vi "packet_build.vi"(9 "D2":u8, 10 "D1":u8, 11 "CMD":u8 format="%x") -> (3 "packet":string)   [LabVIEW 2026]
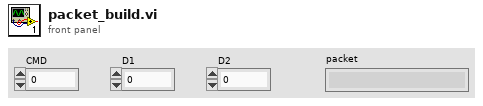
[diagram p1: front panel]
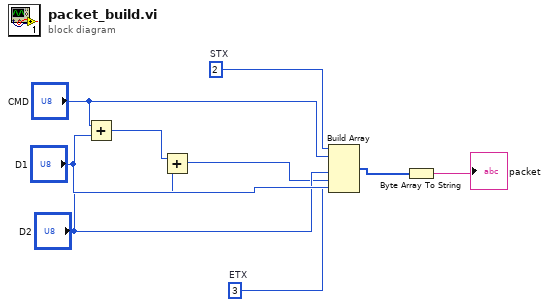
[diagram p0: block diagram]
diagram:
  w3 = u8 3  # ETX
  w8 = u8 2  # STX
  n1 = Add(x="CMD", y="D1") -> (x+y=w9:u8)
  n2 = Add(x=w9, y="D2") -> (x+y=w4:u8)
  n3 = Build Array(w8, "CMD", "D1", "D2", w4, w3) -> (w2:u8[])
  n4 = Byte Array To String(unsigned byte array=w2) -> (string=→"packet":string)
